vi "Migrate - Resolve Entries.vi"(7 "Task Names":string[](array[string]), 8 "error in (no error)":errorcluster, 9 "Project Names":string[](array[string]), 10 "Tasks in":T1, 11 "Projects in":T3) -> (0 "error out":errorcluster, 1 "Project IDs":string[](array[string]), 2 "Tasks out":T1, 3 "Projects out":T3, 4 "Task IDs":string[](array[string]))   [LabVIEW 2024]
doc: "Turns the project and task NAMES of the version-1 entries into IDs. A project that does not exist yet is created with Active = FALSE (and the next Sort Order); a task that does not exist under its project is created the same way. Returns the extended Projects and Tasks and\\2C parallel to the names\\2C the Project IDs and Task IDs.\n\nGenerated by: Claude"
uses:
  Rows/Project.ctl
  Rows/Project List.ctl
  Rows/Task.ctl
  Rows/Task List.ctl
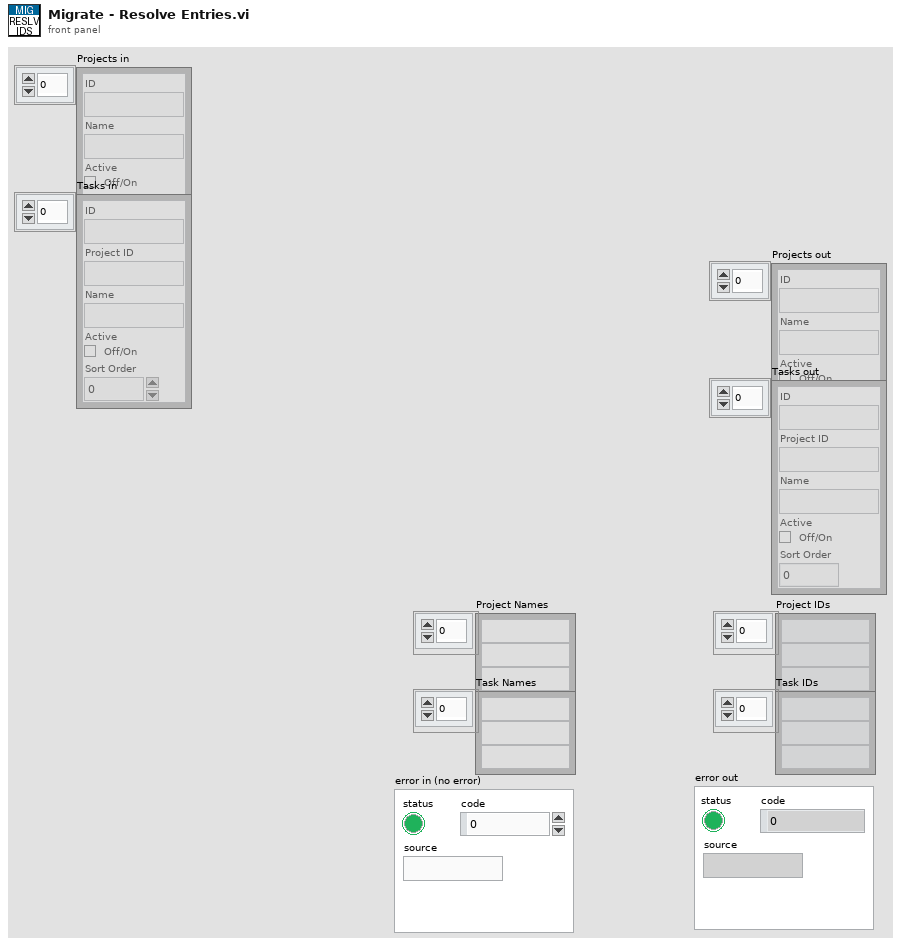
[diagram p1: front panel]
types:
  T1 = typedef "Task List.ctl" = T2[]
  T2 = typedef "Task.ctl" = cluster{"ID":string, "Project ID":string, "Name":string, "Active":bool, "Sort Order":i32}
  T3 = typedef "Project List.ctl" = T4[]
  T4 = typedef "Project.ctl" = cluster{"ID":string, "Name":string, "Active":bool, "Sort Order":i32}
  T5 = cluster{"NI GUID":string, "String":string, "inactive":bool, i32}
  T6 = cluster{"NI GUID":string, "NI GUID":string, "String":string, "inactive":bool, i32}
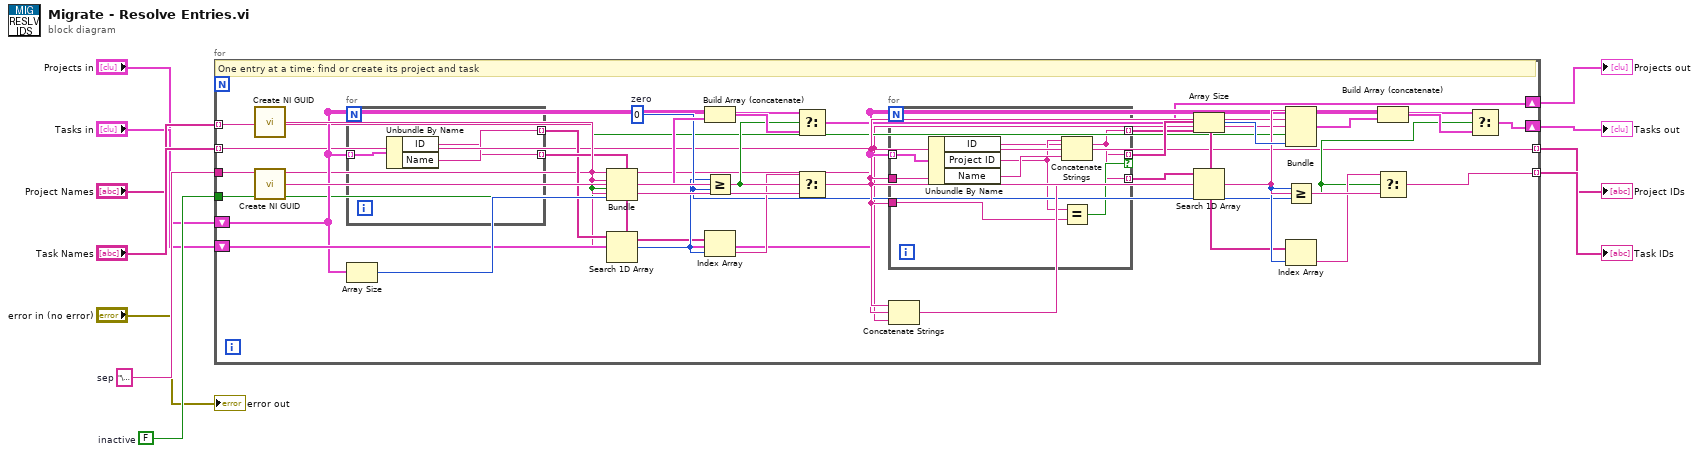
[diagram p0: block diagram]
diagram:
  w7 = FALSE  # inactive
  w6 = "\u0001"  # sep
  n1 = for {
    tunnel: "Project Names" -> [w12] mode=indexing
    tunnel: "Task Names" -> [w13] mode=indexing
    tunnel: w6 -> [w14]
    tunnel: w7 -> [w15]
    shift-right: [w17] -> w8
    shift-left: "Projects in" -> [w16]
    shift-right: [w19] -> w9
    shift-left: "Tasks in" -> [w18]
    tunnel: [w30] -> w10 mode=indexing
    tunnel: [w42] -> w11 mode=indexing
    w23 = 0  # zero
    # "One entry at a time: find or create its project and task"
    n2 = call <vilib>:"Create NI GUID.vi"() -> ("NI GUID"=w26:string)
    n3 = call <vilib>:"Create NI GUID.vi"() -> ("NI GUID"=w38:string)
    n4 = for {
      tunnel: w16 -> [w51] mode=indexing
      tunnel: [w53] -> w20 mode=indexing
      tunnel: [w52] -> w21 mode=indexing
      n5 = Unbundle By Name(w51) -> ("ID"=w52:string, "Name"=w53:string)
    }
    n6 = Array Size(array=w16) -> (size(s)=w27:i32)
    n7 = Bundle("NI GUID"=w26, "String"=w12, "inactive"=w15, w27) -> (w28:T5)  [unwired: 1 in]
    n8 = Search 1D Array(1D array=w20, element=w12) -> (index of element=w22:i32)  [unwired: 1 in]
    n9 = Build Array (concatenate)(w16, w28) -> (w29:T3)
    n10 = Greater Or Equal?(x=w22, y=w23) -> (x >= y?=w24:bool)
    n11 = Index Array(array=w21, index=w22) -> (element=w25:string)
    n12 = Select(t=w16, s=w24, f=w29) -> (s? t:f=w17:T3)
    n13 = Select(t=w25, s=w24, f=w26) -> (s? t:f=w30:string)
    n14 = for {
      tunnel: w18 -> [w43] mode=indexing
      tunnel: w14 -> [w44]
      tunnel: [w46] -> w32 mode=indexing
      tunnel: [w46] -> w33 mode=indexing if=w50
      tunnel: [w49] -> w31 mode=indexing
      tunnel: w30 -> [w45]
      n15 = Unbundle By Name(w43) -> ("ID"=w46:string, "Project ID"=w47:string, "Name"=w48:string)
      n16 = Concatenate Strings(w47, w44, w48) -> (w49:string)
      n17 = Equal?(x=w47, y=w45) -> (x = y?=w50:bool)
    }
    n18 = Concatenate Strings(w30, w14, w13) -> (w34:string)
    n19 = Array Size(array=w33) -> (size(s)=w39:i32)
    n20 = Search 1D Array(1D array=w31, element=w34) -> (index of element=w35:i32)  [unwired: 1 in]
    n21 = Bundle("NI GUID"=w38, "NI GUID"=w30, "String"=w13, "inactive"=w15, w39) -> (w40:T6)  [unwired: 1 in]
    n22 = Greater Or Equal?(x=w35, y=w23) -> (x >= y?=w36:bool)
    n23 = Index Array(array=w32, index=w35) -> (element=w37:string)
    n24 = Build Array (concatenate)(w18, w40) -> (w41:T1)
    n25 = Select(t=w37, s=w36, f=w38) -> (s? t:f=w42:string)
    n26 = Select(t=w18, s=w36, f=w41) -> (s? t:f=w19:T1)
  }
  "Projects out" <- w8
  "Tasks out" <- w9
  "Project IDs" <- w10
  "Task IDs" <- w11
  "error out" <- "error in (no error)"
